vi "read target configuration.vi"(8 "error in":errorcluster, 11 "Targets in":refnum<class "Targets.lvclass">) -> (0 "error out":errorcluster, 2 "Target Configuration":refnum<class "PL_Target Configuration.lvclass">, 3 "Targets out":refnum<class "Targets.lvclass">)   [LabVIEW 2013, in "PL Framework Configuration Tool.lvlib" / "Targets.lvclass"]
uses:
  Targets.lvclass
  Framework Configuration Classes/target configuration/PL_Target Configuration.lvclass
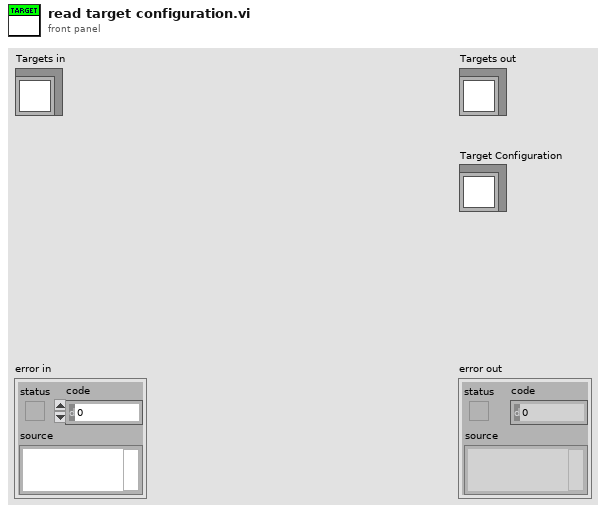
[diagram p1: front panel]
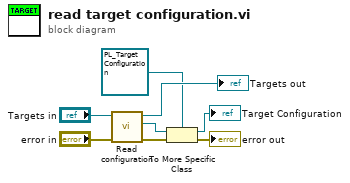
[diagram p0: block diagram]
diagram:
  n1 = call-dynamic "Read configuration.vi"("error in"="error in", "NISE_CEF_serializable node in"="Targets in") -> ("error out"=w8:errorcluster, "configuration"=w5:refnum<class "NISE_CEF_serializable configuration.lvclass">, "NISE_CEF_serializable node out"=→"Targets out":refnum<class "Targets.lvclass">)  [unwired: 7 in]
  n2 = To More Specific Class(target class=refnum<class "PL_Target Configuration.lvclass"> refnum ("Target Configuration"), reference=w5, error in=w8) -> (specific class reference=→"Target Configuration":refnum<class "PL_Target Configuration.lvclass">, error out=→"error out":errorcluster)
